vi "PicoScope2000GetTimebase2.vi"(4 "Number of Samples":u32, 6 "Memory Segment":u32, 7 "Acquisition Settings":T2={"preTriggerSamples"=0, "postTriggerSamples"=1000, "timebase"=2} {"postTriggerSamples" format="%_6p"; "preTriggerSamples" format="%_6p"}, 10 "handle in":i16, 11 "error in (no error)":errorcluster) -> (2 "handle out":i16, 3 "error out":errorcluster, 5 "Properties Panel":T1 {"Max Total Capture Time Available (sec)" format="%.3p"; "Sample Frequency" format="%.3p"; "Sample Rate" format="%.3p"; "Max Samples Available" format="%.3p"; "Total Capture Time (sec)" format="%.3p"})   [LabVIEW 2010]
uses:
  ps2000.dll
  shared/Acquisition Settings.ctl
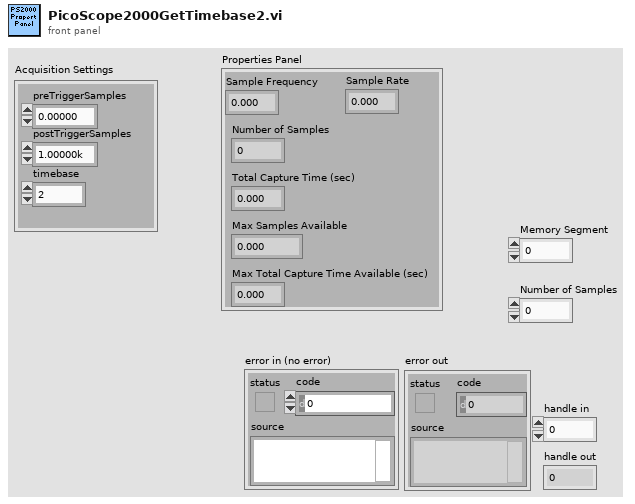
[diagram p1: front panel]
types:
  T1 = cluster{"Sample Frequency":sgl, "Sample Rate":sgl, "Max Samples Available":i32, "Number of Samples":u32, "Total Capture Time (sec) ":sgl, "Max Total Capture Time Available (sec)":sgl}
  T2 = typedef "Acquisition Settings.ctl" = cluster{"preTriggerSamples":u64, "postTriggerSamples":u64, "timebase":u32}
  T3 = cluster{sgl, sgl, "maxSamples":i32, "Number of Samples":u32, sgl, sgl}
  T4 = cluster{sgl, sgl, "max_sample":i32, "Number of Samples":u32, sgl, sgl}
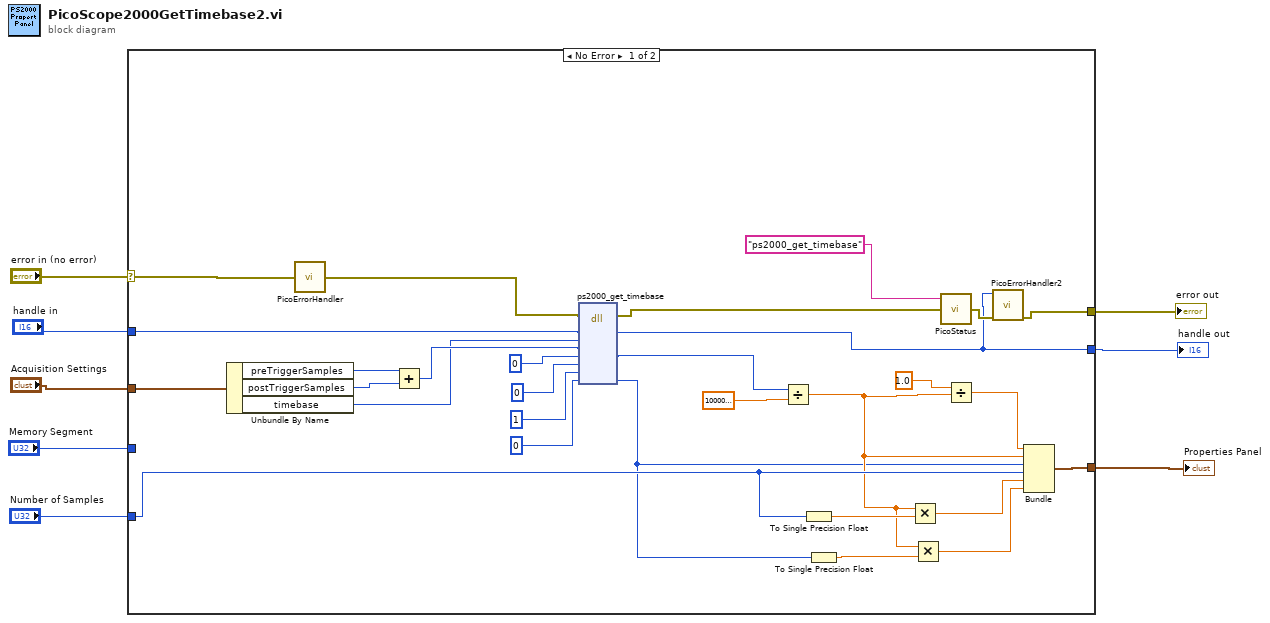
[diagram p0: block diagram]
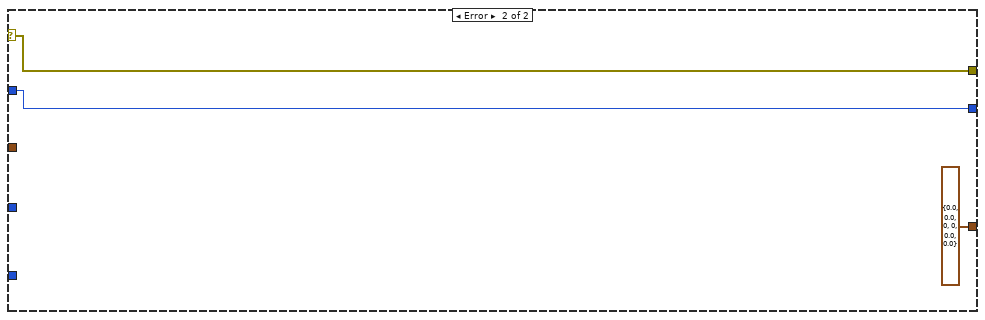
[diagram p2: hidden frame]
diagram:
  n1 = case shown="No Error" "error in (no error)" {
    selector: "error in (no error)" -> [w33 w40]
    tunnel: [w21 w40] -> w8
    tunnel: [w10 w39] -> w7
    tunnel: "Memory Segment" -> [_ _]
    tunnel: "Number of Samples" -> [w29 _]
    tunnel: "handle in" -> [w18 w39]
    tunnel: "Acquisition Settings" -> [w32 _]
    tunnel: [w26 T3 {0.0, 0.0, "maxSamples"=0, "Number of Samples"=0, 0.0, 0.0}] -> w1
    frame No Error {
      n2 = Unbundle By Name(w32) -> ("preTriggerSamples"=w35:u64, "postTriggerSamples"=w36:u64, "timebase"=w16:u32)
      n3 = call "PicoErrorHandler.vi"("error in"=w33) -> ("error out"=w19:errorcluster)
      n4 = Add(x=w35, y=w36) -> (x+y=w17:u64)
      n5 = dll-call lib="PS2000.dll" fn="ps2000_get_timebase"(error in=w19, "handle"=w18, "timebase"=w16, "no_of_samples"=w17, "time_interval_ms"=0, "time_units"=i16 0, "oversample"=i16 1, "max_sample"=0 ("maxSamples")) -> (error out=w11:errorcluster, "handle"=w10:i16, "time_interval_ms"=w9:i32, "max_sample"=w20:i32)  [unwired: 7 in, 1 out]
      n6 = Divide(x=w9, y=sgl 1000000000.0) -> (x/y=w25:sgl)
      n7 = To Single Precision Float(number=w29) -> (single precision float=w31:sgl)
      n8 = To Single Precision Float(number=w20) -> (single precision float=w28:sgl)
      n9 = Multiply(x=w25, y=w31) -> (x*y=w30:sgl)
      n10 = Multiply(x=w25, y=w28) -> (x*y=w27:sgl)
      n11 = call "PicoStatus.vi"("error in"=w11, "source"="ps2000_get_timebase") -> ("error out"=w22:errorcluster)  [unwired: 1 in]
      n12 = Divide(x=sgl 1.0, y=w25) -> (x/y=w23:sgl)
      n13 = call "PicoErrorHandler2.vi"("error in (no error)"=w22, "handle In"=w10) -> ("error out"=w21:errorcluster)  [unwired: 9 in]
      n14 = Bundle(w23, w25, "max_sample"=w20, "Number of Samples"=w29, w30, w27) -> (w26:T4)  [unwired: 1 in]
    }
    frame Error {
    }
  }
  "error out" <- w8
  "handle out" <- w7
  "Properties Panel" <- w1
